vi "stop helper loop.vi"(8 "错误输入（无错误）":errorcluster, 11 "helper loop data":T1) -> (0 "错误输出":errorcluster)   [LabVIEW 2025, in "XButton.lvlib" / "button3.xctl"]
uses:
  button3.xctl
  helper loop Events.ctl
  move event.ctl
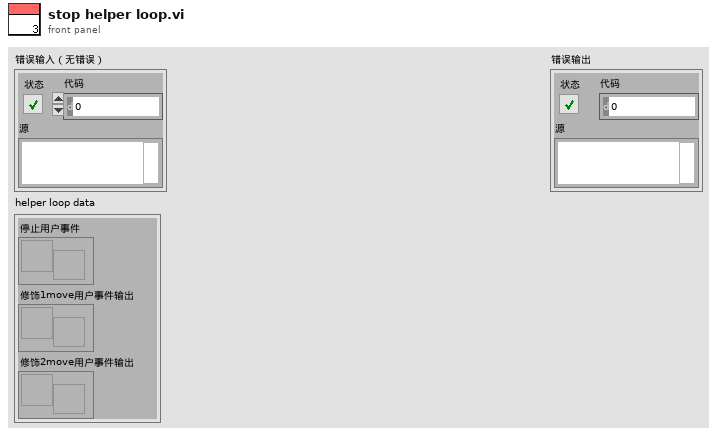
[diagram p1: front panel]
types:
  T1 = typedef "XButton.lvlib/button3.xctl/helper loop Events.ctl" = cluster{"停止用户事件":refnum<user-event>, "修饰1move用户事件输出":refnum<user-event>, "修饰2move用户事件输出":refnum<user-event>}
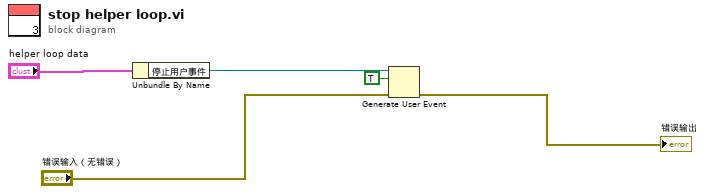
[diagram p0: block diagram]
diagram:
  n1 = Unbundle By Name("helper loop data") -> ("停止用户事件"=w5:refnum<user-event>)
  n2 = Generate User Event(user event=w5, event data cluster=TRUE ("事件数据"), error in="错误输入（无错误）") -> (error out=→"错误输出":errorcluster)  [unwired: 1 in, 1 out]
